vi "RemoteVI Parse Arguments.vi"(0 "args":string[](array[string])) -> (4 "options":T1={"share"="", "port"=8100, "token"="", "whole network"=FALSE, "view only"=FALSE, "landing port"=8088})   [LabVIEW 2020, in "RemoteVI.lvlib"]
doc: "RemoteVI Server.exe's command line (the arguments after --, as Application:Command Line Arguments returns them without the program): --share <window title> shares that window at start; --port N its port (default 8100); --token T its token (default: random); --whole-network and --view-only as the check boxes; --landing-port P the landing page's port (default 8088, 0 = no landing page). Unknown arguments and a last flag without its value are ignored; a value that is not a number from 0 to 65535 keeps the default. Pure. Reference: parseArgs() in tools\\lib\\server-app.mjs."
uses:
  RemoteVI.lvlib
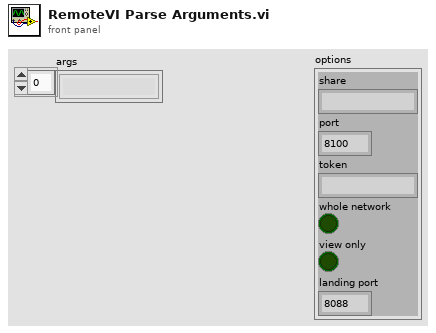
[diagram p1: front panel]
types:
  T1 = cluster{"share":string, "port":u16, "token":string, "whole network":bool, "view only":bool, "landing port":u16}
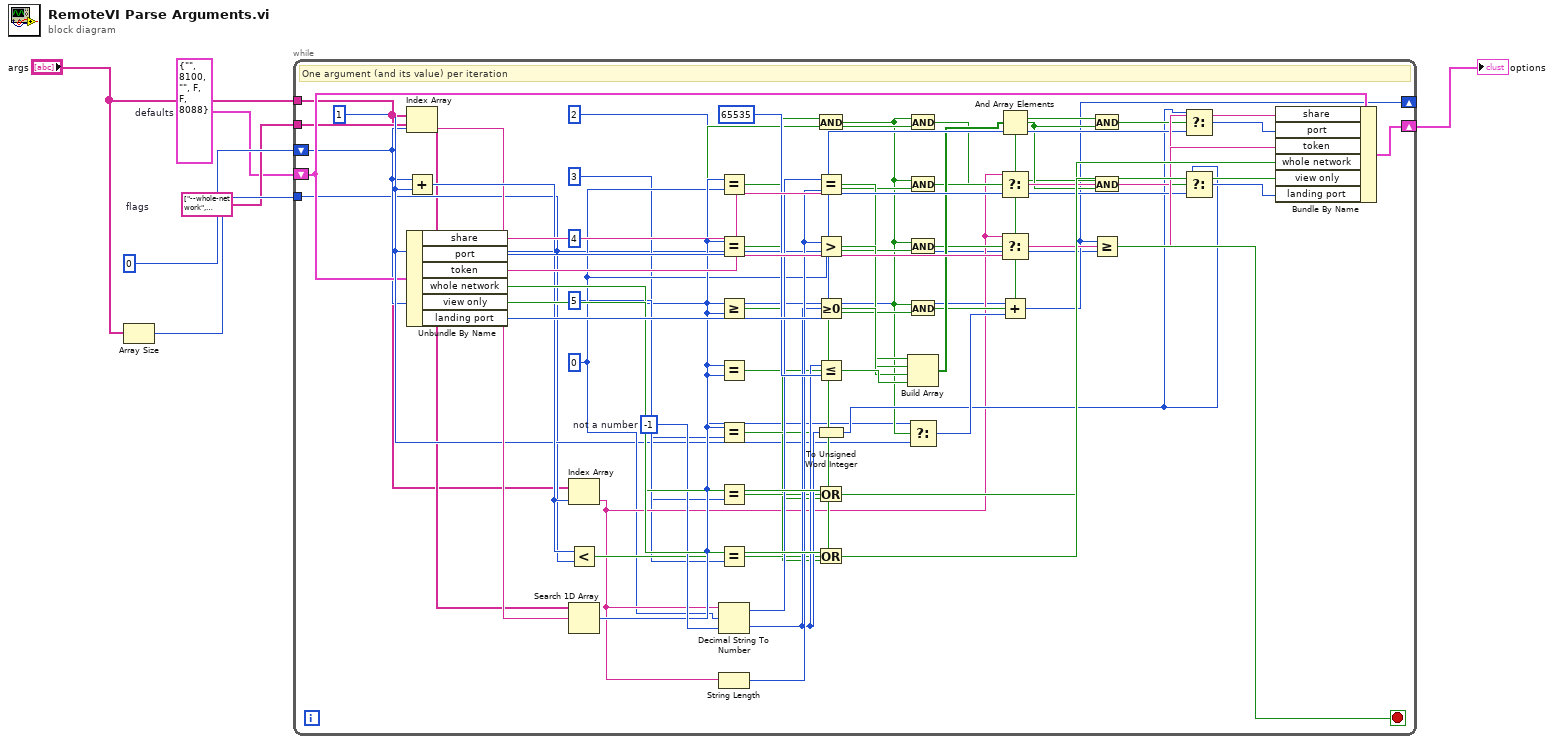
[diagram p0: block diagram]
diagram:
  w3 = string[] ["--whole-network", "--view-only", "--share", "--port", "--token", "--landing-port"]  # flags
  w2 = T1 {"share"="", "port"=8100, "token"="", "whole network"=FALSE, "view only"=FALSE, "landing port"=8088}  # defaults
  n1 = Array Size(array="args") -> (size(s)=w4:i32)
  n2 = while {
    tunnel: "args" -> [w7]
    tunnel: w3 -> [w8]
    shift-right: [w11] -> _
    shift-left: 0 -> [w10]
    shift-right: [w13] -> w6
    shift-left: w2 -> [w12]
    tunnel: w4 -> [w9]
    stop <- w64 stop-if-true
    w37 = -1  # not a number
    w19 = 0
    w15 = 2
    w14 = 1
    # "One argument (and its value) per iteration"
    n3 = Index Array(array=w7, index=w10) -> (element=w20:string)
    n4 = Add(x=w10, y=w14) -> (x+y=w21:i32)
    n5 = Unbundle By Name(w12) -> ("share"=w51:string, "port"=w52:u16, "token"=w53:string, "whole network"=w54:bool, "view only"=w55:bool, "landing port"=w56:u16)
    n6 = Index Array(array=w7, index=w21) -> (element=w22:string)
    n7 = Less?(x=w21, y=w9) -> (x < y?=w23:bool)
    n8 = Search 1D Array(1D array=w8, element=w20) -> (index of element=w24:i32)  [unwired: 1 in]
    n9 = Equal?(x=w24, y=w19) -> (x = y?=w25:bool)
    n10 = Equal?(x=w24, y=w14) -> (x = y?=w26:bool)
    n11 = Greater Or Equal?(x=w24, y=w15) -> (x >= y?=w27:bool)
    n12 = Equal?(x=w24, y=w15) -> (x = y?=w29:bool)
    n13 = Equal?(x=w24, y=3) -> (x = y?=w30:bool)
    n14 = Equal?(x=w24, y=4) -> (x = y?=w31:bool)
    n15 = Equal?(x=w24, y=5) -> (x = y?=w32:bool)
    n16 = Decimal String To Number(string=w22, offset=w19, default (0L)=w37) -> (offset past number=w38:i32, number=w39:i32)
    n17 = String Length(string=w22) -> (length=w40:i32)
    n18 = And(x=w27, y=w23) -> (x .and. y?=w28:bool)
    n19 = Equal?(x=w38, y=w40) -> (x = y?=w41:bool)
    n20 = Greater?(x=w40, y=w19) -> (0:w42:bool)
    n21 = Greater Or Equal To 0?(x=w39) -> (x >= 0?=w43:bool)
    n22 = Less Or Equal?(x=w39, y=65535) -> (x <= y?=w45:bool)
    n23 = To Unsigned Word Integer(number=w39) -> (unsigned 16bit integer=w48:u16)
    n24 = Or(x=w54, y=w25) -> (x .or. y?=w61:bool)
    n25 = Or(x=w55, y=w26) -> (x .or. y?=w62:bool)
    n26 = And(x=w28, y=w29) -> (x .and. y?=w33:bool)
    n27 = And(x=w28, y=w30) -> (x .and. y?=w34:bool)
    n28 = And(x=w28, y=w31) -> (x .and. y?=w35:bool)
    n29 = And(x=w28, y=w32) -> (x .and. y?=w36:bool)
    n30 = Build Array(w41, w42, w43, w45) -> (w46:bool[])
    n31 = Select(t=w15, s=w28, f=w14) -> (s? t:f=w63:i32)
    n32 = And Array Elements(Boolean array=w46) -> (logical AND=w47:bool)
    n33 = Select(t=w22, s=w33, f=w51) -> (s? t:f=w57:string)
    n34 = Select(t=w22, s=w35, f=w53) -> (s? t:f=w58:string)
    n35 = Add(x=w10, y=w63) -> (x+y=w11:i32)
    n36 = And(x=w34, y=w47) -> (x .and. y?=w49:bool)
    n37 = And(x=w36, y=w47) -> (x .and. y?=w50:bool)
    n38 = Greater Or Equal?(x=w11, y=w9) -> (x >= y?=w64:bool)
    n39 = Select(t=w48, s=w49, f=w52) -> (s? t:f=w59:u16)
    n40 = Select(t=w48, s=w50, f=w56) -> (s? t:f=w60:u16)
    n41 = Bundle By Name(cluster=w12, "share"=w57, "port"=w59, "token"=w58, "whole network"=w61, "view only"=w62, "landing port"=w60) -> (w13:T1)
  }
  "options" <- w6
